vi "Modify Template.vi"(8 "error in":errorcluster, 11 "ILabVIEWFile in":refnum<class "Type Definition.lvclass">) -> (0 "error out":errorcluster, 3 "ILabVIEWFile out":refnum<class "Type Definition.lvclass">)   [LabVIEW 2026, in "Type Definition.lvclass"]
doc: "This method modifies (i.e. adds/removes/replaces elements in the template) to implement the current file."
uses:
  Type Definition.lvclass
  Type Definition.lvclass/Type Definition.ctl
  Interfaces/IElement/IElement.lvclass
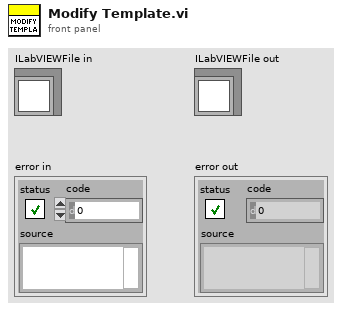
[diagram p1: front panel]
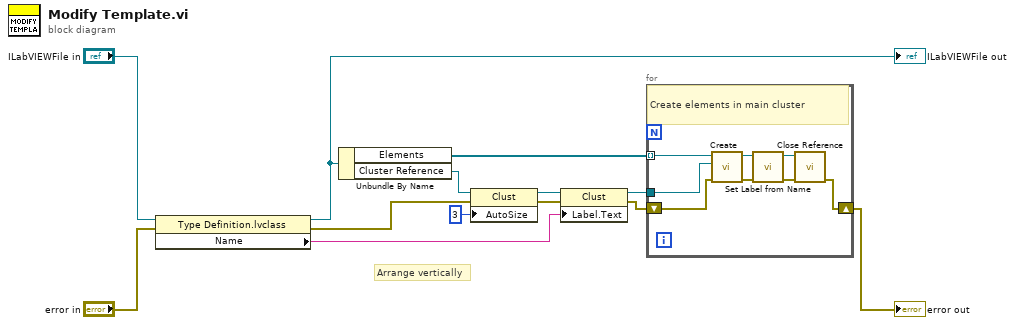
[diagram p0: block diagram]
diagram:
  # "Arrange vertically"
  n1 = property class="Type Definition.lvclass"(reference="ILabVIEWFile in", error in="error in") -> (reference out=w2:refnum<class "Type Definition.lvclass">, error out=w10:errorcluster, "Name"=w1:string)
  "ILabVIEWFile out" <- w2
  n2 = Unbundle By Name(w2) -> ("Elements"=w5:refnum<class "IElement.lvclass">[], "Cluster Reference"=w6:refnum<vi>)
  n3 = property on="Property Node" class="Clust"(reference=w6, error in=w10, "AutoSize"=u32 3 ("Auto Sizing")) -> (reference out=w7:refnum<vi>, error out=w13:errorcluster)
  n4 = property on="Property Node" class="Clust"(reference=w7, error in=w13, "Label.Text"=w1) -> (reference out=w4:refnum<vi>, error out=w12:errorcluster)
  n5 = for {
    tunnel: w5 -> [w17] mode=indexing
    tunnel: w4 -> [w14]
    shift-right: [w18] -> w11
    shift-left: w12 -> [w21]
    # "Create elements in main cluster"
    n6 = call-dynamic "Create.vi"("error in"=w21, "Parent Reference"=w14, "IElement in"=w17) -> ("error out"=w19:errorcluster, "IElement out"=w16:refnum<class "IElement.lvclass">)  [unwired: 7 in]
    n7 = call-dynamic "Set Label from Name.vi"("error in"=w19, "IElement in"=w16) -> ("error out"=w20:errorcluster, "IElement out"=w15:refnum<class "IElement.lvclass">)  [unwired: 8 in]
    n8 = call-dynamic "Close Reference.vi"("error in"=w20, "IElement in"=w15) -> ("error out"=w18:errorcluster)  [unwired: 8 in, 1 out]
  }
  "error out" <- w11
